vi "InitializeRectanglesByIndex.vi"(8 "error in (no error)":errorcluster, 10 "Rectangles":string[](array[string]), 11 "Setting Database in":refnum<class "Setting Database.lvclass">) -> (0 "error out":errorcluster, 3 "Setting Database out":refnum<class "Setting Database.lvclass">)   [LabVIEW 2019, in "Setting Database.lvclass"]
uses:
  Setting Database.lvclass
  Rectangle Settings/Rectangle Settings.lvclass
  C:/Users/Albro/Documents/GitHub/AFM-Lithography/lvsrc/Classes/Settings/ObjectSettings/ObjectSettings.lvclass
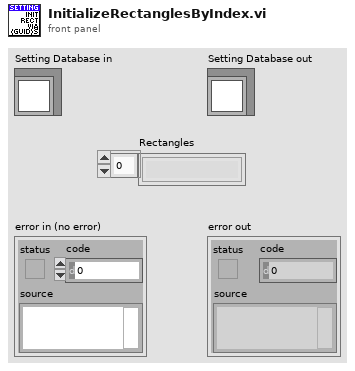
[diagram p1: front panel]
types:
  T1 = cluster{"Path":string, "Funnel":string, "Rectangle":string, "Dot":string}
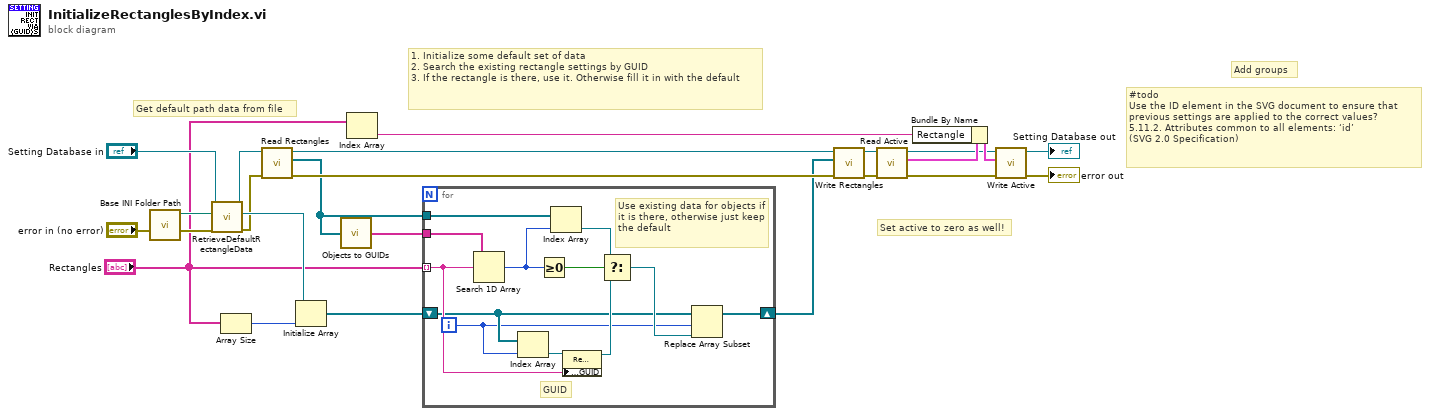
[diagram p0: block diagram]
diagram:
  # "Get default path data from file"
  # "Set active to zero as well!"
  # "1. Initialize some default set of data\n2. Search the existing rectangle settings by GUID\n3. If the rectangle is there, use it. Otherwise fill it in with the default"
  # "Add groups"
  # "#todo\nUse the ID element in the SVG document to ensure that previous settings are applied to the correct values? \n5.11.2. Attributes common to all elements: ‘id’ \n(SVG 2.0 Specification)"
  n1 = call "Base INI Folder Path.vi"() -> ("Base Path"=w23:path)  [unwired: 11 in]
  n2 = call "RetrieveDefaultRectangleData.vi"("error in (no error)"="error in (no error)", "Path"=w23, "Setting Database In"="Setting Database in") -> ("error out"=w16:errorcluster, "Rectangle Settings.lvclass"=w21:refnum<class "Rectangle Settings.lvclass">, "Setting Database Out"=w22:refnum<class "Setting Database.lvclass">)  [unwired: 6 in]
  n3 = Array Size(array="Rectangles") -> (size(s)=w10:i32)
  n4 = call "Read Rectangles.vi"("error in (no error)"=w16, "Setting Database in"=w22) -> ("error out"=w19:errorcluster, "Rectangles"=w6:refnum<class "Rectangle Settings.lvclass">[], "Setting Database out"=w17:refnum<class "Setting Database.lvclass">)  [unwired: 7 in]
  n5 = Initialize Array(w21, w10) -> (w4:refnum<class "Rectangle Settings.lvclass">[])
  n6 = call "Objects to GUIDs.vi"("Objects"=w6) -> ("GUIDs"=w5:string[])  [unwired: 3 in, 1 out]
  n7 = Index Array(array="Rectangles") -> (element=w1:string)  [unwired: 1 in]
  n8 = for {
    tunnel: w6 -> [w33]
    shift-right: [w35] -> w3
    shift-left: w4 -> [w25]
    tunnel: w5 -> [w32]
    tunnel: "Rectangles" -> [w30] mode=indexing
    i -> [w24]
    # "GUID"
    # "Use existing data for objects if it is there, otherwise just keep the default"
    n9 = Search 1D Array(1D array=w32, element=w30) -> (index of element=w34:i32)  [unwired: 1 in]
    n10 = Index Array(array=w25, index=w24) -> (element=w31:refnum<class "Rectangle Settings.lvclass">)
    n11 = Greater Or Equal To 0?(x=w34) -> (x >= 0?=w29:bool)
    n12 = Index Array(array=w33, index=w34) -> (element=w28:refnum<class "Rectangle Settings.lvclass">)
    n13 = property class="Rectangle Settings.lvclass"(reference=w31, "Accessors:GUID"=w30) -> (reference out=w26:refnum<class "Rectangle Settings.lvclass">)  [unwired: 1 in, 1 out]
    n14 = Select(t=w28, s=w29, f=w26) -> (s? t:f=w27:refnum<class "Rectangle Settings.lvclass">)
    n15 = Replace Array Subset(array=w25, new element=w27, index=w24) -> (w35:refnum<class "Rectangle Settings.lvclass">[])
  }
  n16 = call "Write Rectangles.vi"("error in (no error)"=w19, "Rectangles"=w3, "Setting Database in"=w17) -> ("error out"=w20:errorcluster, "Setting Database out"=w18:refnum<class "Setting Database.lvclass">)  [unwired: 7 in]
  n17 = call "Read Active.vi"("error in (no error)"=w20, "Setting Database in"=w18) -> ("error out"=w13:errorcluster, "Active"=w14:T1, "Setting Database out"=w12:refnum<class "Setting Database.lvclass">)  [unwired: 7 in]
  n18 = Bundle By Name(cluster=w14, "Rectangle"=w1) -> (w15:T1)
  n19 = call "Write Active.vi"("error in (no error)"=w13, "Active"=w15, "Setting Database in"=w12) -> ("error out"=→"error out":errorcluster, "Setting Database out"=→"Setting Database out":refnum<class "Setting Database.lvclass">)  [unwired: 7 in]
